vi "Explorer Path.vi"(8 "error in (no error)":errorcluster, 10 "Explorer Path":path, 11 "Bar in":refnum<class "Bar.lvclass">) -> (0 "error out":errorcluster, 3 "Bar out":refnum<class "Bar.lvclass">)   [LabVIEW 2015, in "Simple Progress Bar.lvlib" / "Bar.lvclass"]
doc: "Enable the Explore button in the progress bar user interface so the user can browse process files result. The directory of the <b>Explorer Path</b> must exist on disk."
uses:
  Class/Bar.lvclass
  Class/Bar.lvclass/Bar.ctl
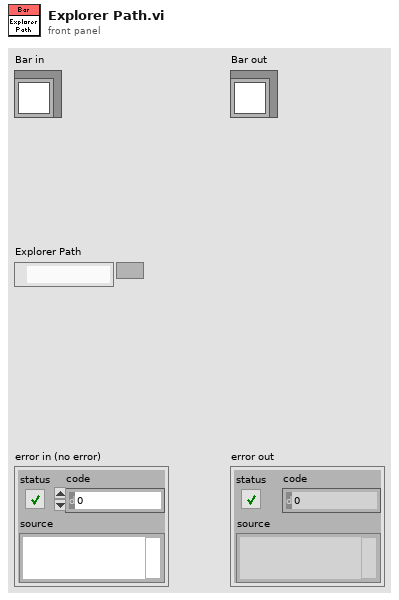
[diagram p1: front panel]
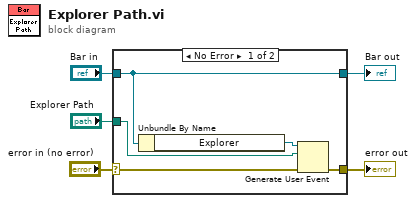
[diagram p0: block diagram]
diagram:
  n1 = case shown="No Error" "error in (no error)" {
    selector: "error in (no error)" -> [w9 w11]
    tunnel: "Bar in" -> [w7 w12]
    tunnel: [w7 w12] -> w3
    tunnel: [w8 w11] -> w2
    tunnel: "Explorer Path" -> [w6 _]
    frame No Error {
      n2 = Unbundle By Name(w7) -> ("Explorer"=w10:refnum<user-event>)
      n3 = Generate User Event(user event=w10, event data cluster=w6, error in=w9) -> (error out=w8:errorcluster)  [unwired: 1 in, 1 out]
    }
    frame Error {
    }
  }
  "error out" <- w2
  "Bar out" <- w3
